vi "Unload Plot.vi"(8 "error in (no error)":errorcluster, 10 "Plot Index":i32, 11 "Data Viewer in":refnum<class "Data Viewer.lvclass">) -> (0 "error out":errorcluster, 3 "Data Viewer out":refnum<class "Data Viewer.lvclass">)   [LabVIEW 2020, in "Data Viewer.lvlib" / "Data Viewer.lvclass"]
uses:
  Data Viewer.lvclass
  Data Serie--cluster.ctl
  Data Viewer.lvclass/Data Viewer.ctl
  Data Viewer.lvlib
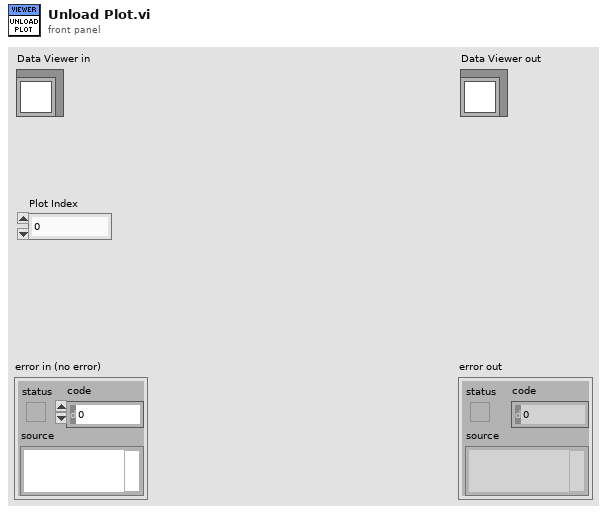
[diagram p1: front panel]
types:
  T1 = typedef "Data Viewer.lvlib/Data Serie--cluster.ctl" = cluster{"Name":string, "Unit":string, "Sample Rate[Hz]":dbl, "Delta t[S]":dbl, "t0":timestamp, "Length":i32, "Time":timestamp[], "Value":dbl[]}
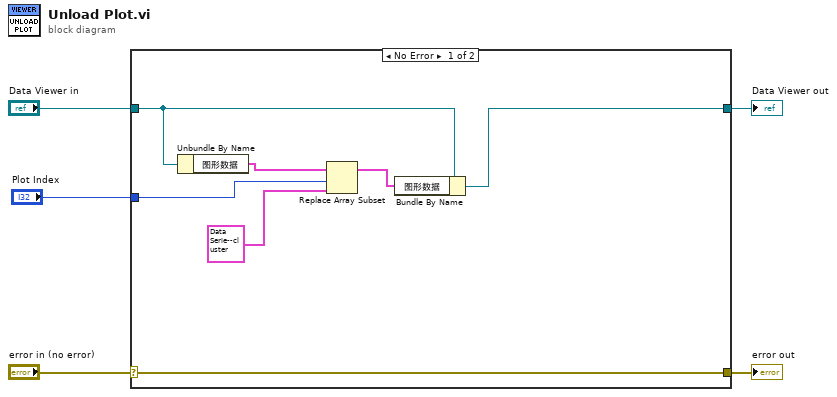
[diagram p0: block diagram]
diagram:
  n1 = case shown="No Error" "error in (no error)" {
    selector: "error in (no error)" -> [w12 w14]
    tunnel: [w12 w14] -> w4
    tunnel: [w7 w13] -> w2
    tunnel: "Data Viewer in" -> [w11 w13]
    tunnel: "Plot Index" -> [w9 _]
    frame No Error {
      n2 = Unbundle By Name(w11) -> ("图形数据"=w10:T1[])
      n3 = Replace Array Subset(array=w10, new element=T1 {"Name"="", "Unit"="", "Sample Rate[Hz]"=0.0, "Delta t[S]"=0.0, "t0"=timestamp(0 s since 1904-01-01), "Length"=0, "Time"=[], "Value"=[]} ("new element/subarray"), index=w9) -> (w6:T1[])
      n4 = Bundle By Name(cluster=w11, "图形数据"=w6) -> (w7:refnum<class "Data Viewer.lvclass">)
    }
    frame Error {
    }
  }
  "error out" <- w4
  "Data Viewer out" <- w2
